vi "Data entry form.vi"(0 "Stack in":refnum<class "Stack.lvclass">, 1 "Adhesive type":string, 2 "Temperature (C)":string, 3 "Relative humidity":string, 5 "Position":dbl, 7 "Module Type":string="CMU,LD,Full,200,CuW", 9 "Module?":bool, 11 "error in (no error)":errorcluster, 12 "Operator":string, 13 "ROC version":string) -> (4 "Stack out":refnum<class "Stack.lvclass">, 8 "Cancelled?":bool, 15 "error out":errorcluster)   [LabVIEW 2021, in "Stack.lvclass"]
uses:
  Stack.lvclass
  Stack.lvclass/Stack.ctl
panel:
  in  "Is real run":bool
  in  "Tape Batch (optional)":string
  out "Time":string
  in  "?":string="Scan module QR code for real runs. For dummy runs leave empty."
  in  "Module stack name (no hyphens; include 320)":string
  in  "Cancel Button":bool
  in  "Comments":string
  in  "?":string="Leave Base/Top Layer ID fields empty for dummy runs!!"
  in  "?":string="Record sensor visual inspection comments here."
  out "Sensor thickness":string
  out "BP Type":string
  out "Geometry":string
  in  "Baselayer thickness for glue dispense":dbl
  out "Resolution":string
  out "Date":string
  in  "Glue Batch":string
  in  "Component Tray ID":string
  in  "Assembly Tray ID":string
  in  "PUT ID":string
  in  "Baselayer ID":string
  in  "Toplayer ID":string
  in  "Submit":bool
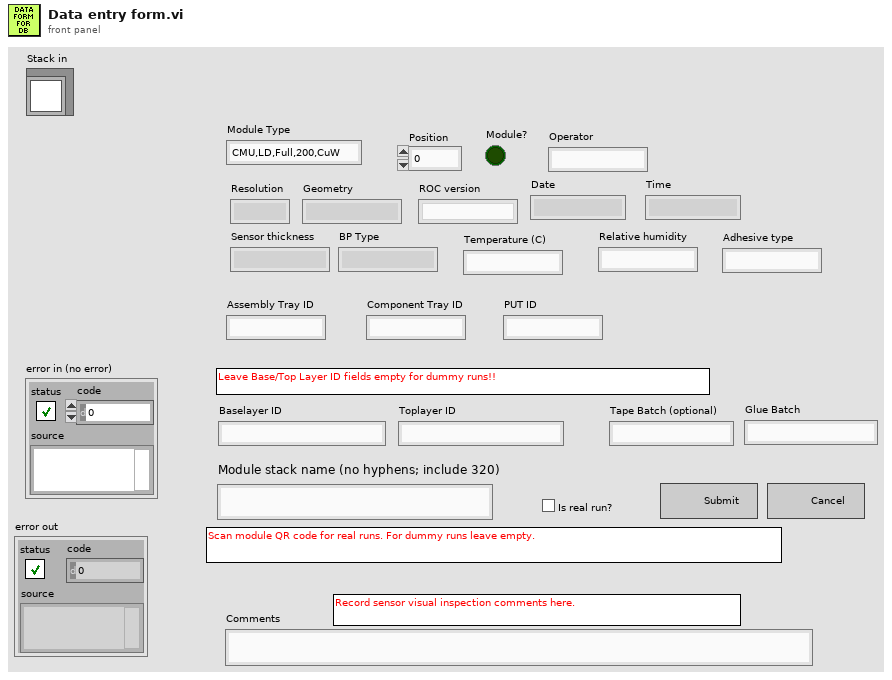
[diagram p1: front panel]
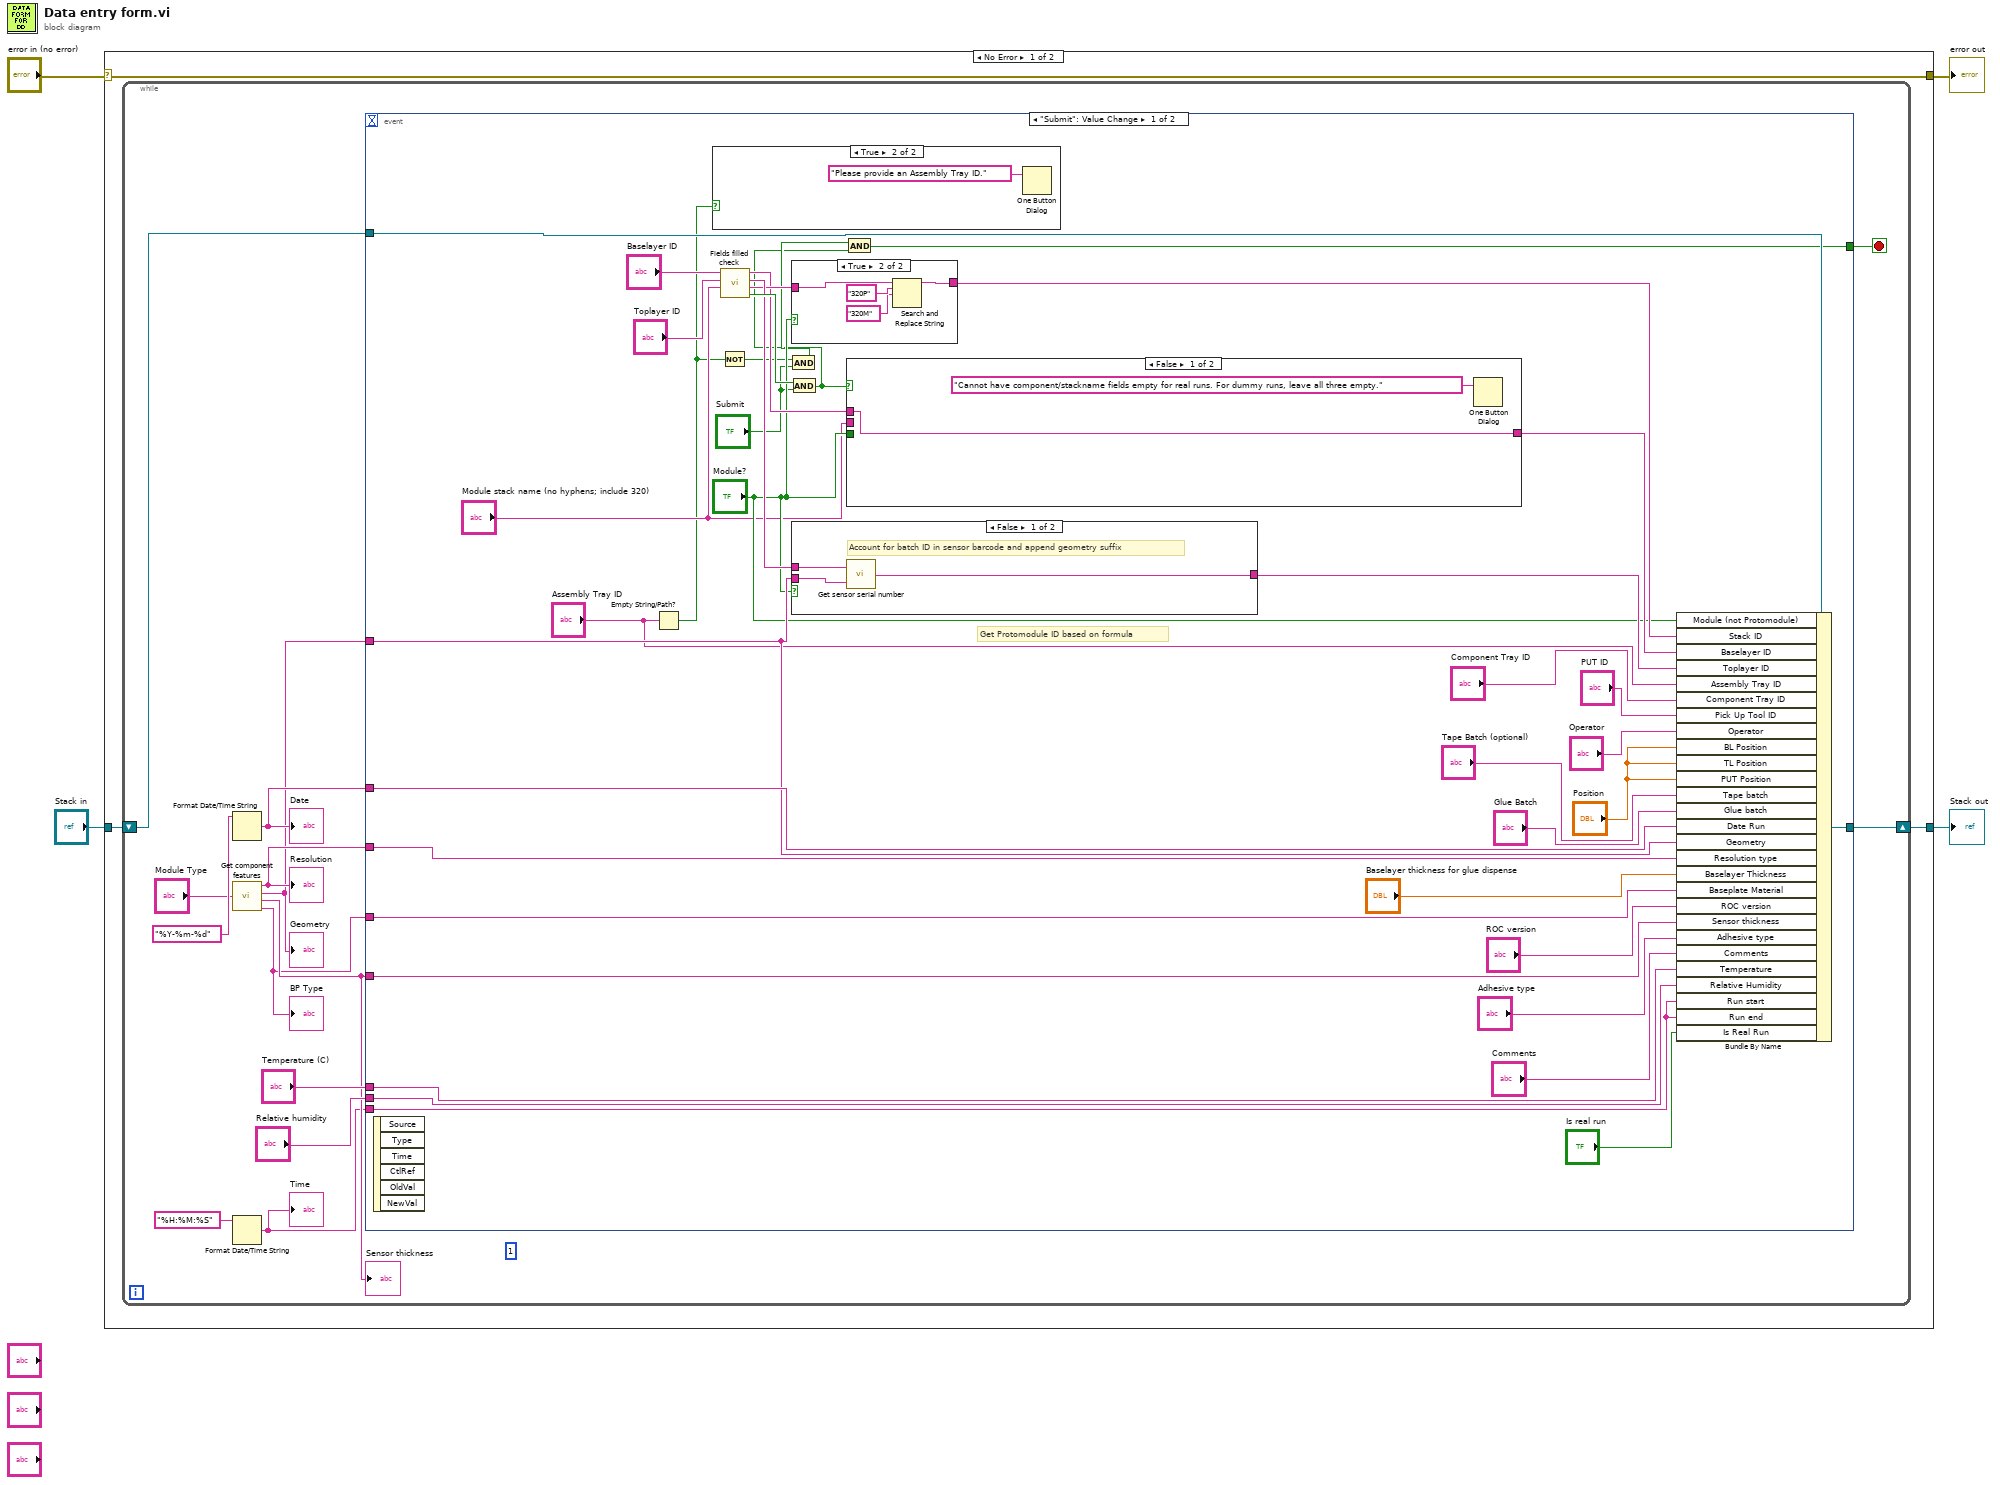
[diagram p0: block diagram]
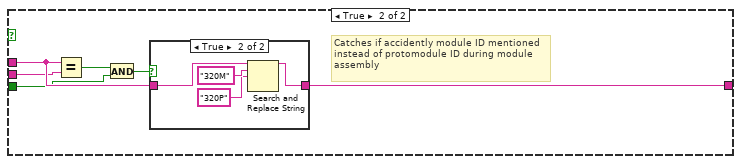
[diagram p3: hidden frame]
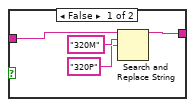
[diagram p5: hidden frame]
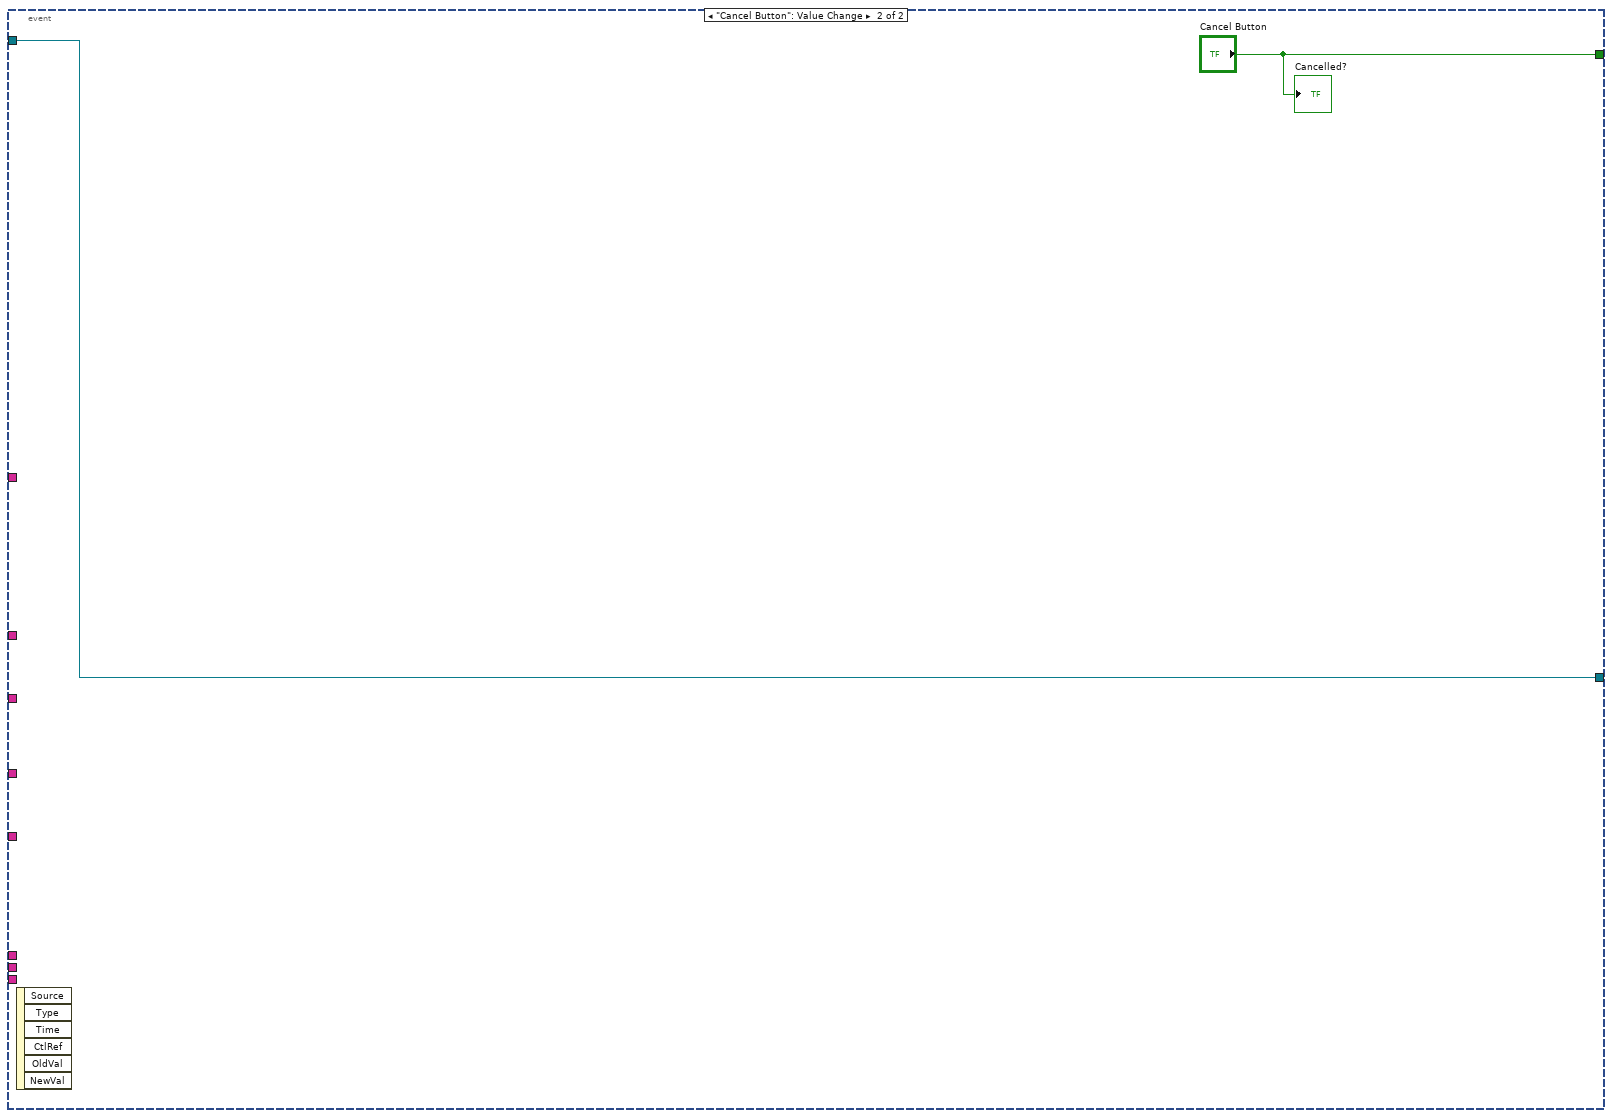
[diagram p7: hidden frame]
diagram:
  n1 = case shown="No Error" "error in (no error)" {
    selector: "error in (no error)" -> [w7 w90]
    tunnel: [w7 w90] -> w3
    tunnel: [w5 w89] -> w1
    tunnel: "Stack in" -> [w6 w89]
    frame No Error {
      n2 = while {
        shift-right: [w21] -> w5
        shift-left: w6 -> [w15]
        stop <- w16 stop-if-true
        (unwired) 1 ("offset (0)")
        n3 = Format Date/Time String(time format string (%c)="%Y-%m-%d") -> (date/time string=w19:string)  [unwired: 2 in]
        "Date" <- w19
        n4 = call "Get component features.vi"("Module Type"="Module Type") -> ("Resolution"=w13:string, "Geometry"=w12:string, "Sensor thickness"=w11:string, "BP Type"=w10:string)  [unwired: 1 in, 1 out]
        "Resolution" <- w13
        "Geometry" <- w12
        "BP Type" <- w10
        "Sensor thickness" <- w11
        n5 = Format Date/Time String(time format string (%c)="%H:%M:%S") -> (date/time string=w8:string)  [unwired: 2 in]
        "Time" <- w8
        n6 = event shown="[0] \"Submit\": Value Change" {
          selector: _ -> [_ _]
          dyn-events: _ -> [_ _]
          timeout: _ -> [_ _]
          tunnel: w15 -> [w60 w88]
          tunnel: [w56 w88] -> w21
          tunnel: w13 -> [w52 _]
          tunnel: w10 -> [w51 _]
          tunnel: w11 -> [w50 _]
          tunnel: w19 -> [w49 _]
          tunnel: w12 -> [w39 _]
          tunnel: "Temperature (C)" -> [w47 _]
          tunnel: "Relative humidity" -> [w46 _]
          tunnel: [w23 "Cancel Button"] -> w16
          tunnel: w8 -> [w38 _]
          event "Submit": Value Change {
            # "Get Protomodule ID based on formula"
            n7 = event-data() -> ()  [unwired: 1 in, 6 out]
            n8 = Empty String/Path?(string/path="Assembly Tray ID") -> (empty?=w28:bool)
            n9 = case shown="True" w28 {
              frame False {
              }
              frame True {
                n10 = One Button Dialog(message="Please provide an Assembly Tray ID.") -> ()  [unwired: 1 in, 1 out]
              }
            }
            n11 = call "Fields filled check.vi"("Module stack name (no hyphens; include 320)"="Module stack name (no hyphens; include 320)", "Toplayer ID"="Toplayer ID", "Baselayer ID"="Baselayer ID") -> ("Fields fully (not)filled"=w42:bool, "Module stack name (no hyphens; include 320) out"=w40:string, "Toplayer ID out"=w41:string, "Baselayer ID  out"=w32:string)  [unwired: 1 in]
            n12 = Not(x=w28) -> (.not. x?=w27:bool)
            n13 = And(x=w27, y="Submit") -> (x .and. y?=w26:bool)
            n14 = And(x=w42, y="Submit") -> (x .and. y?=w24:bool)
            n15 = case shown="True" "Module?" {
              tunnel: w40 -> [w76 w80]
              tunnel: [w75 w79] -> w45
              frame False {
                n16 = Search and Replace String(input string=w76, search string="320M", replace string="320P" ("replace string (\"\")")) -> (result string=w75:string)  [unwired: 5 in, 3 out]
              }
              frame True {
                n17 = Search and Replace String(input string=w80, search string="320P", replace string="320M" ("replace string (\"\")")) -> (result string=w79:string)  [unwired: 5 in, 3 out]
              }
            }
            n18 = case shown="False" "Module?" {
              tunnel: w39 -> [w84 _]
              tunnel: w41 -> [w85 w86]
              tunnel: [w83 w86] -> w48
              frame False {
                # "Account for batch ID in sensor barcode and append geometry suffix"
                n19 = call "Get sensor serial number.vi"("Geometry"=w84, "Toplayer ID"=w85) -> ("Toplayer ID out"=w83:string)
              }
              frame True {
              }
            }
            n20 = And(x=w26, y=w24) -> (x .and. y?=w23:bool)
            n21 = case shown="False" w24 {
              tunnel: w32 -> [w62 w68]
              tunnel: [w62 w69] -> w31
              tunnel: "Module?" -> [_ w65]
              tunnel: "Module stack name (no hyphens; include 320)" -> [_ w67]
              frame False {
                n22 = One Button Dialog(message="Cannot have component/stackname fields empty for real runs. For dummy runs, leave all three empty.") -> ()  [unwired: 1 in, 1 out]
              }
              frame True {
                # "Catches if accidently module ID mentioned instead of protomodule ID during module assembly"
                n23 = Equal?(x=w68, y=w67) -> (x = y?=w66:bool)
                n24 = And(x=w66, y=w65) -> (x .and. y?=w64:bool)
                n25 = case shown="True" w64 {
                  tunnel: w68 -> [w70 w72]
                  tunnel: [w70 w71] -> w69
                  frame False {
                  }
                  frame True {
                    n26 = Search and Replace String(input string=w72, search string="320M", replace string="320P" ("replace string (\"\")")) -> (result string=w71:string)  [unwired: 5 in, 3 out]
                  }
                }
              }
            }
            n27 = Bundle By Name(cluster=w60, "Module (not Protomodule)"="Module?", "Stack ID"=w45, "Baselayer ID"=w31, "Toplayer ID"=w48, "Assembly Tray ID"="Assembly Tray ID", "Component Tray ID"="Component Tray ID", "Pick Up Tool ID"="PUT ID", "Operator"="Operator", "BL Position"="Position", "TL Position"="Position", "PUT Position"="Position", "Tape batch"="Tape Batch (optional)", "Glue batch"="Glue Batch", "Date Run"=w49, "Geometry"=w39, "Resolution type"=w52, "Baselayer Thickness"="Baselayer thickness for glue dispense", "Baseplate Material"=w51, "ROC version"="ROC version", "Sensor thickness"=w50, "Adhesive type"="Adhesive type", "Comments"="Comments", "Temperature"=w47, "Relative Humidity"=w46, "Run start"=w38, "Run end"=w38, "Is Real Run"="Is real run") -> (w56:refnum<class "Stack.lvclass">)
          }
          event "Cancel Button": Value Change {
            n28 = event-data() -> ()  [unwired: 1 in, 6 out]
            "Cancelled?" <- "Cancel Button"
          }
        }
      }
    }
    frame Error {
    }
  }
  "error out" <- w3
  "Stack out" <- w1
